vi "SMTP Email MIME Send File Attachment.vi"(4 "MIME content-type":string caption="type de contenu MIME", 5 "translit":string, 6 "binary (F)":bool caption="binaire (F)", 7 "character set":string caption="jeu de caractères", 8 "error in (no error)":errorcluster caption="entrée d'erreur (pas d'erreur)", 9 "name (file name)":string caption="nom (nom du fichier)", 10 "path":path caption="chemin", 11 "smtp session":T1 caption="session smtp") -> (0 "error out":errorcluster caption="sortie d'erreur", 2 "file error":errorcluster caption="erreur de fichier", 3 "smtp session out":T1 caption="session smtp en sortie")   [LabVIEW 2022 SP3, in "Copie de NI_SMTPEmail.lvlib"]
uses:
  Copie de NI_SMTPEmail.lvlib
  SMTP Email Session.ctl
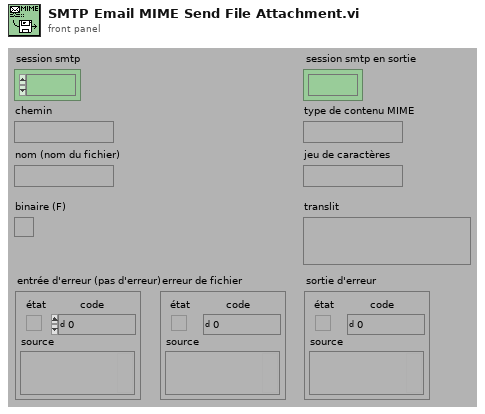
[diagram p1: front panel]
types:
  T1 = typedef "Copie de NI_SMTPEmail.lvlib/SMTP Email Session.ctl" = refnum<k1>
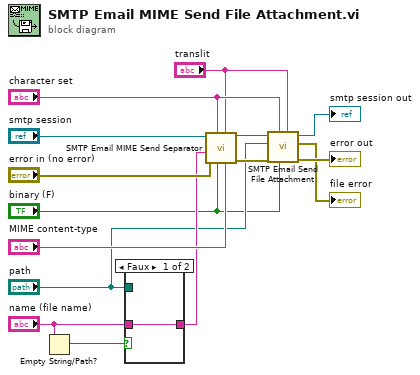
[diagram p0: block diagram]
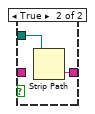
[diagram p2: hidden frame]
diagram:
  n1 = Empty String/Path?(string/path="name (file name)") -> (empty?=w12:bool)
  n2 = case shown="Faux" w12 {
    tunnel: "name (file name)" -> [w16 _]
    tunnel: [w16 w18] -> w11
    tunnel: "path" -> [_ w17]
    frame False {
    }
    frame True {
      n3 = Strip Path(path=w17) -> (name=w18:string)  [unwired: 1 out]
    }
  }
  n4 = call "SMTP Email MIME Send Separator.vi"("MIME content-type"="MIME content-type", "translit"="translit", "binary (F)"="binary (F)", "character set"="character set", "error in (no error)"="error in (no error)", "name"=w11, "smtp session"="smtp session") -> ("error out"=w9:errorcluster, "smtp session out"=w7:T1)  [unwired: 3 in]
  n5 = call "SMTP Email Send File Attachment.vi"("translit"="translit", "binary? (F)"="binary (F)", "character set"="character set", "error in (no error)"=w9, "path"="path", "smtp session"=w7) -> ("error out"=→"error out":errorcluster, "file error"=→"file error":errorcluster, "smtp session out"=→"smtp session out":T1)  [unwired: 3 in]
